vi "upload.vi"(8 "error in":errorcluster, 10 "File":path, 11 "Nominal Client in":refnum<class "Nominal Client.lvclass">) -> (0 "error out":errorcluster, 2 "Path to S3 File":string, 3 "Nominal Client out":refnum<class "Nominal Client.lvclass">)   [LabVIEW 2020, in "Nominal Client.lvclass"]
doc: "Uploads a file to Nominal by taking the file path as input and automatically selecting the appropriate upload technique based on the file size. Small files are uploaded in a single operation, while large files are uploaded using a multipart strategy for efficiency and reliability."
uses:
  Nominal Client.lvclass
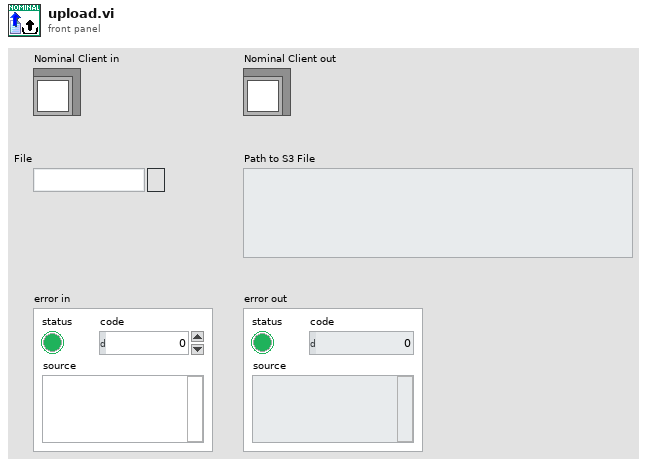
[diagram p1: front panel]
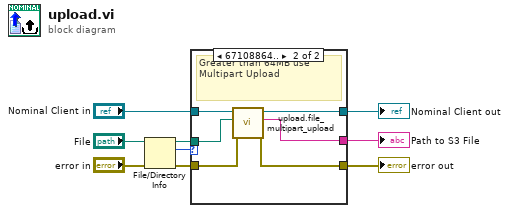
[diagram p0: block diagram]
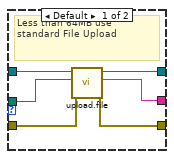
[diagram p2: hidden frame]
diagram:
  n1 = File/Directory Info(path="File", error in="error in") -> (path out=w6:path, size=w8:i64, error out=w3:errorcluster)  [unwired: 4 out]
  n2 = case shown="67108864.." w8 {
    tunnel: w6 -> [w15 w18]
    tunnel: "Nominal Client in" -> [w14 w21]
    tunnel: [w13 w20] -> w4
    tunnel: w3 -> [w12 w17]
    tunnel: [w11 w16] -> w2
    tunnel: [w10 w19] -> w1
    frame Default {
      # "Less than 64MB use standard File Upload"
      n3 = call "upload.file.vi"("error in"=w12, "File"=w15, "Nominal Client in"=w14) -> ("error out"=w11:errorcluster, "Path to S3 File"=w10:string, "Nominal Client out"=w13:refnum<class "Nominal Client.lvclass">)  [unwired: 6 in]
    }
    frame 67108864.. {
      # "Greater than 64MB use Multipart Upload"
      n4 = call "upload.file_multipart_upload.vi"("error in"=w17, "File Path"=w18, "Nominal Client in"=w21) -> ("error out"=w16:errorcluster, "S3 Path to File"=w19:string, "Nominal Client out"=w20:refnum<class "Nominal Client.lvclass">)  [unwired: 6 in]
    }
  }
  "Nominal Client out" <- w4
  "error out" <- w2
  "Path to S3 File" <- w1
